vi "Tester.vi"() -> ()   [LabVIEW 2025]
uses:
  VarexWrapper.lvlib
panel:
  in  "loop delay (ms)":u32=5
  in  "Stop":bool
  out "Image Out":T1(plugin-control)
  out "serialNumber out":string
  out "model out":string
  out "channelType out":string
  out "error out":errorcluster
  out "lib-version":string
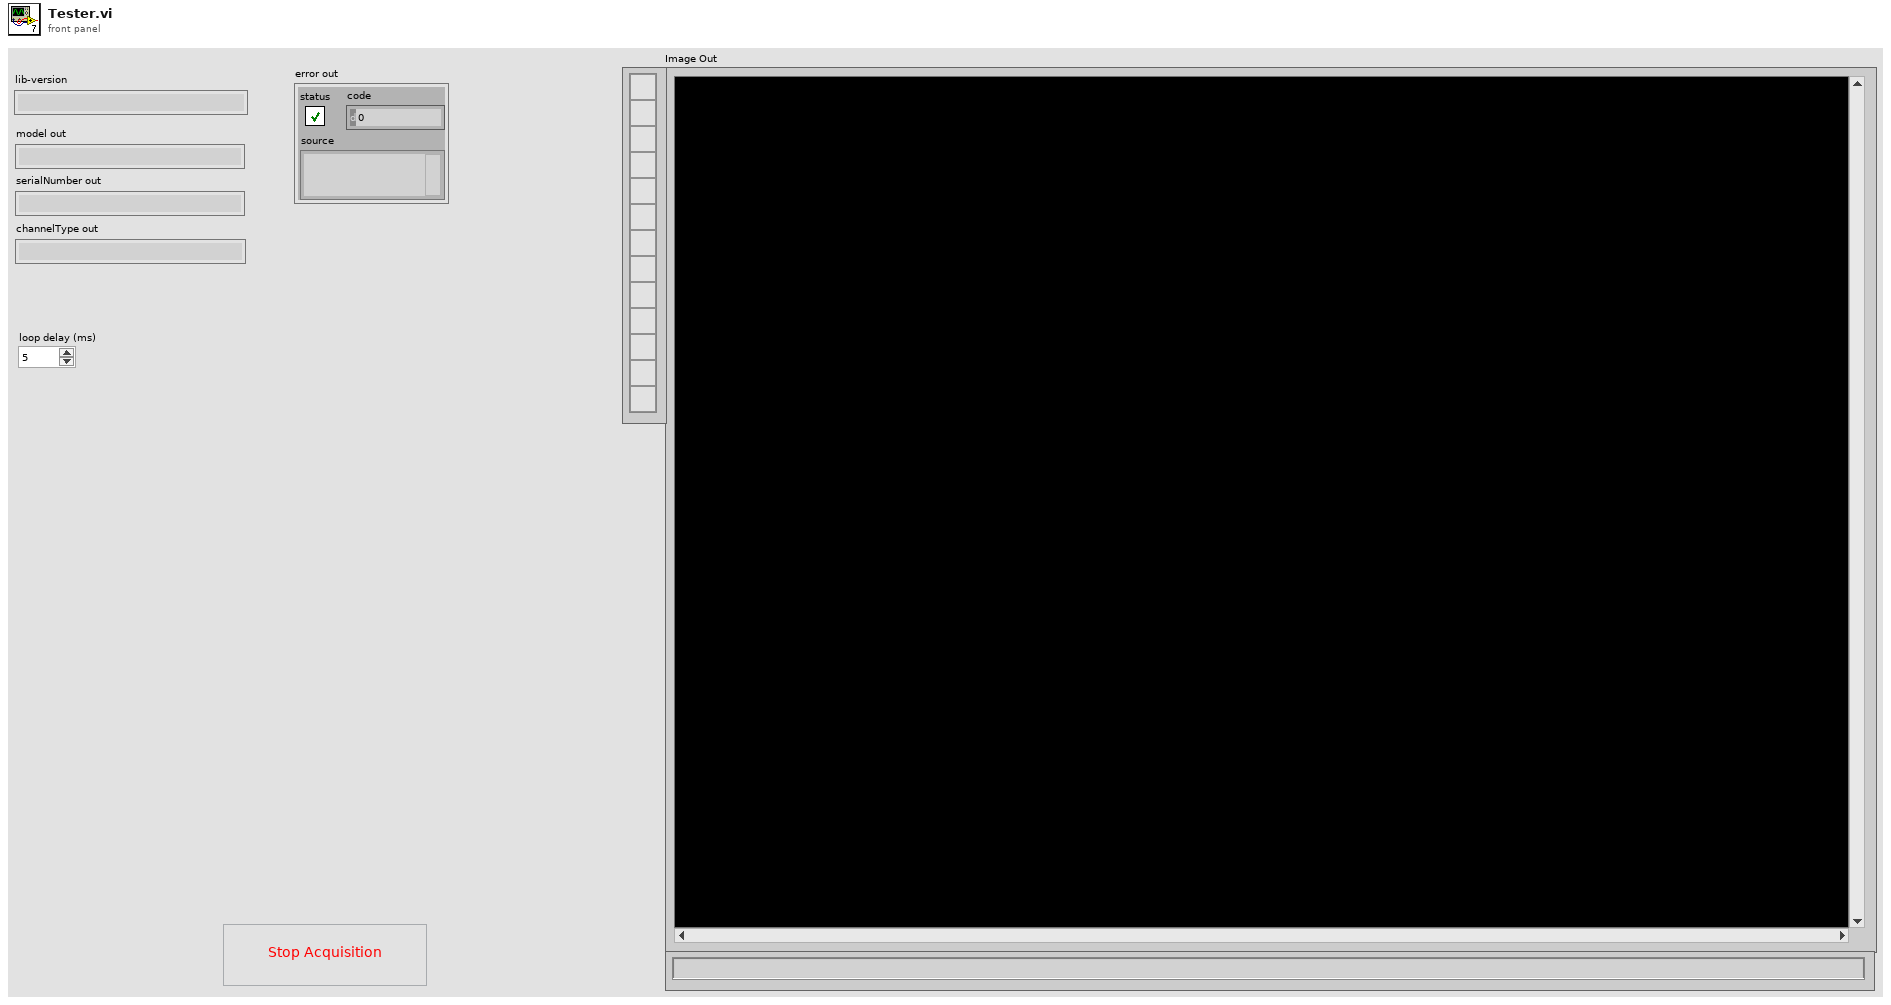
[diagram p1: front panel]
types:
  T1 = typedef "IMAQ Image.ctl" = refnum<image>
  T2 = typedef "Image Type" = u32
  T3 = enum32{"Map Pixel Pointer", "Unmap Pixel Pointer", "Get Pixels Infos"}
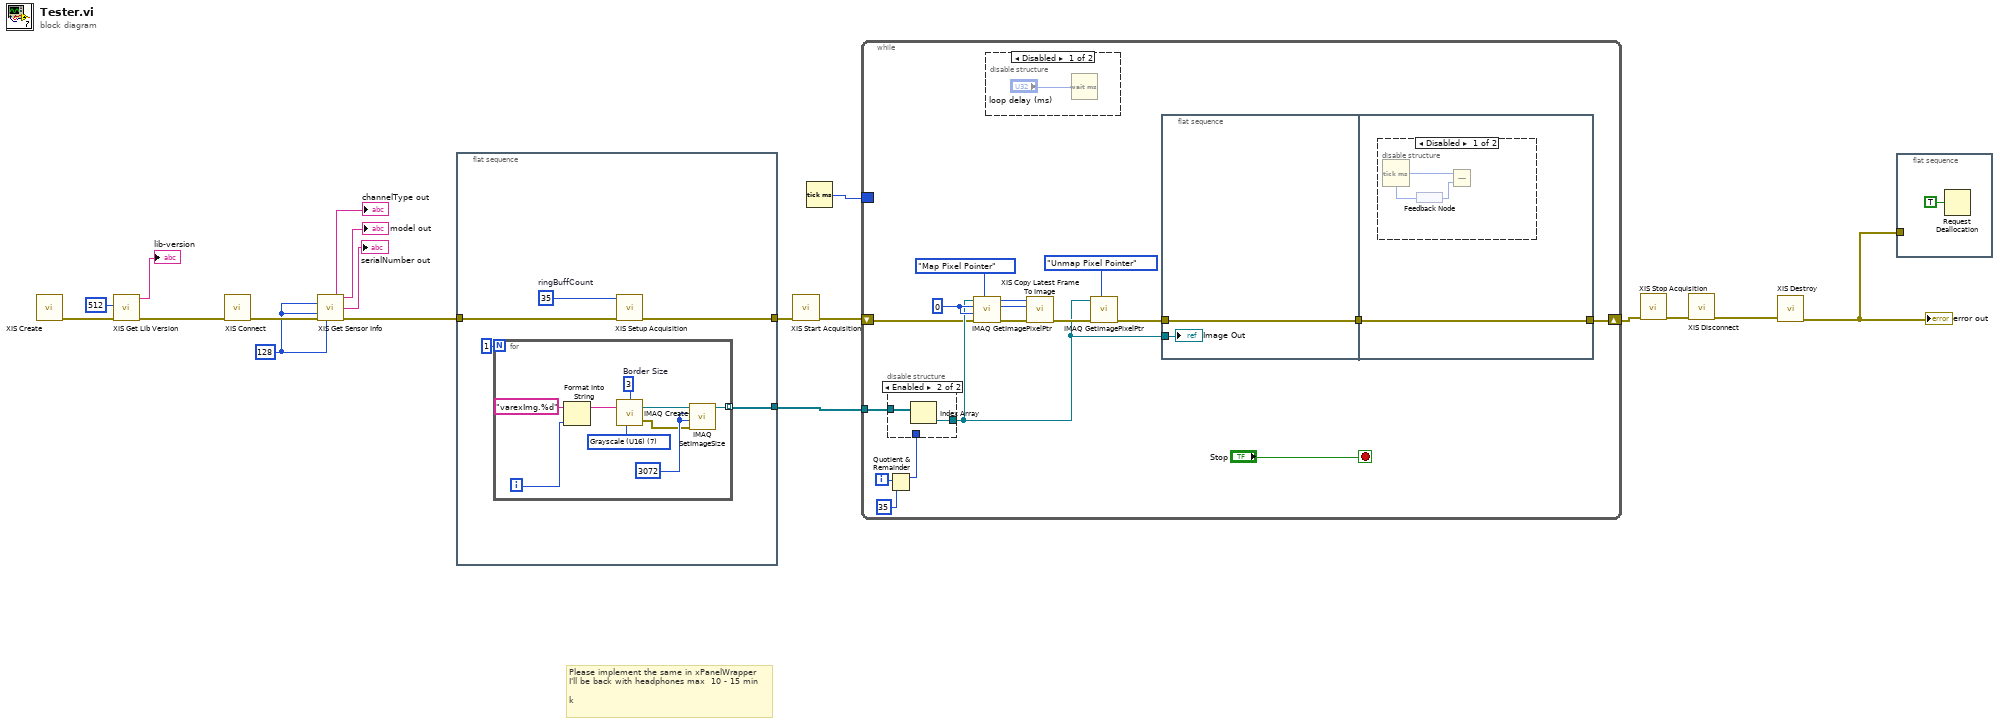
[diagram p0: block diagram]
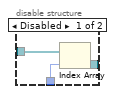
[diagram p3: hidden frame]
diagram:
  w10 = 128 ("modelSize")
  # "Please implement the same in xPanelWrapper\nI'll be back with headphones max  10 - 15 min\n\nk"
  n1 = call "XIS Create.vi"() -> ("error out"=w18:errorcluster)  [unwired: 10 in, 1 out]
  n2 = call "XIS Get Lib Version.vi"("error in (no error)"=w18, "bufferSize"=512) -> ("error out"=w17:errorcluster, "buffer out"=→"lib-version":string)  [unwired: 7 in, 1 out]
  n3 = call "XIS Connect.vi"("error in (no error)"=w17) -> ("error out"=w14:errorcluster)  [unwired: 9 in, 1 out]
  n4 = call "XIS Get Sensor Info.vi"("modelSize"=w10, "serialNumberSize"=w10, "error in (no error)"=w14, "channelTypeSize"=w10) -> ("channelType out"=→"channelType out":string, "model out"=→"model out":string, "serialNumber out"=→"serialNumber out":string, "error out"=w1:errorcluster)  [unwired: 7 in, 1 out]
  n5 = flat-sequence {
    tunnel: w1 -> [w23]
    tunnel: [w22] -> w9
    tunnel: [w20] -> w4
    frame #0 {
      w21 = 35  # ringBuffCount
      n6 = for {
        N: 1 -> [_]
        tunnel: [w29] -> w20 mode=indexing
        i -> [w24]
        w27 = 3  # Border Size
        w28 = 3072 ("X Resolution")
        w31 = T2 7 items=["Grayscale (U8)", "Grayscale (I16)", "Grayscale (SGL)", "Complex (CSG)", "RGB (U32)", "HSL (U32)", "RGB (U64)", "Grayscale (U16)"] ("Image Type")
        n7 = Format Into String(initial string="varexImg.%d" ("Image Name"), w24) -> (resulting string=w25:string)  [unwired: 2 in, 1 out]
        n8 = call "IMAQ Create"("Border Size"=w27, "Image Name"=w25, "Image Type"=w31) -> ("New Image"=w30:T1, "error out"=w26:errorcluster)  [unwired: 2 in]
        n9 = call "IMAQ SetImageSize"("error in (no error)"=w26, "Y Resolution"=w28, "X Resolution"=w28, "Image"=w30) -> ("Image Out"=w29:T1)  [unwired: 1 in, 1 out]
      }
      n10 = call "XIS Setup Acquisition.vi"("error in (no error)"=w23, "ringBuffCount"=w21) -> ("error out"=w22:errorcluster)  [unwired: 8 in, 1 out]
    }
  }
  n11 = call "XIS Start Acquisition.vi"("error in (no error)"=w9) -> ("error out"=w8:errorcluster)  [unwired: 9 in, 1 out]
  n12 = Tick Count (ms)() -> (millisecond timer value=w3:u32)
  n13 = while {
    shift-right: [w41] -> w7
    shift-left: w8 -> [w33]
    tunnel: w4 -> [w38]
    border: w3 -> [_]
    i -> [w37]
    stop <- "Stop" stop-if-true
    w44 = 0 ("X Coordinate")
    n14 = Quotient & Remainder(x=w37, y=35) -> (x-y*floor(x/y)=w35:i32)  [unwired: 1 out]
    n15 = disable-structure shown="Enabled" {
      disable-tunnel: w38 -> [w53 w55]
      disable-tunnel: w35 -> [w52 _]
      disable-tunnel: [w51 w54] -> w34
      frame Disabled {
        n16 = Index Array(array=w53, index=w52) -> (element=w51:T1)
      }
      frame Enabled {
        n17 = Index Array(array=w55) -> (element=w54:T1)  [unwired: 1 in]
      }
    }
    n18 = call "IMAQ GetImagePixelPtr"("Function"=T3."Map Pixel Pointer", "error in (no error)"=w33, "Y Coordinate"=w44, "X Coordinate"=w44, "Image"=w34) -> ("error out"=w45:errorcluster, "LineWidth(Pixels)"=w47:i32, "Pixel Pointer out"=w48:u64)  [unwired: 1 in, 3 out]
    n19 = disable-structure shown="Disabled" {
      frame Disabled {
        n20 = Wait (ms)(milliseconds to wait="loop delay (ms)") -> ()  [unwired: 1 out]
      }
      frame Enabled {
      }
    }
    n21 = call "XIS Copy Latest Frame To Image.vi"("error in (no error)"=w45, "LVLineWidthPixels"=w47, "LVImagePtr"=w48) -> ("error out"=w46:errorcluster)  [unwired: 7 in, 1 out]
    n22 = call "IMAQ GetImagePixelPtr"("Function"=T3."Unmap Pixel Pointer", "error in (no error)"=w46, "Image"=w34) -> ("error out"=w42:errorcluster)  [unwired: 3 in, 5 out]
    n23 = flat-sequence {
      tunnel: w42 -> [w57]
      tunnel: w34 -> [w56]
      tunnel: [w57] -> w39
      tunnel: [w58] -> w41
      tunnel: w39 -> [w58]
      frame #0 {
        "Image Out" <- w56
      }
      frame #1 {
        n24 = disable-structure shown="Disabled" {
          frame Disabled {
            n25 = Tick Count (ms)() -> (millisecond timer value=w59:u32)
            n26 = feedback #1() -> (w60:u32)
            n27 = feedback-in #1(w59) -> ()
            n28 = Subtract(x=w59, y=w60) -> (x-y=w61:u32)
          }
          frame Enabled {
          }
        }
      }
    }
  }
  n29 = call "XIS Stop Acquisition.vi"("error in (no error)"=w7) -> ("error out"=w6:errorcluster)  [unwired: 9 in, 1 out]
  n30 = call "XIS Disconnect.vi"("error in (no error)"=w6) -> ("error out"=w5:errorcluster)  [unwired: 9 in, 1 out]
  n31 = call "XIS Destroy.vi"("error in (no error)"=w5) -> ("error out"=w2:errorcluster)  [unwired: 9 in, 1 out]
  "error out" <- w2
  n32 = flat-sequence {
    tunnel: w2 -> [_]
    frame #0 {
      n33 = Request Deallocation(TRUE ("flag")) -> ()
    }
  }
